vi "VIH HelpGen - HTML - Build A HREF Tag to File.vi"(7 "HTML Folder":path, 8 "file status":enum16{"unknown", "good", "bad"}(ring), 10 "Referenced HTML File":path, 11 "Name":string) -> (0 "file status out":enum16{"unknown", "good", "bad"}(ring), 2 "dup Referenced HTML File":path, 3 "HTML out":string)   [LabVIEW 2014]
doc: "::: VI Helpeks :::\nCopyright (c) 2000-2026 Konstantin Shifershteyn. All rights reserved."
panel:
  # "VI Helpeks\nCopyright (c) 2012-2026 Konstantin Shifershteyn"
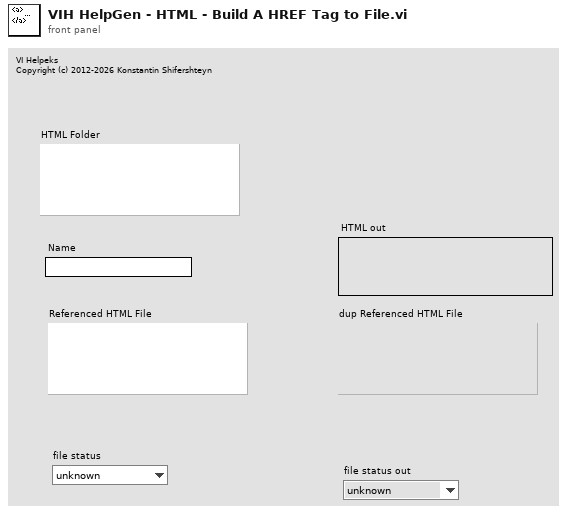
[diagram p1: front panel]
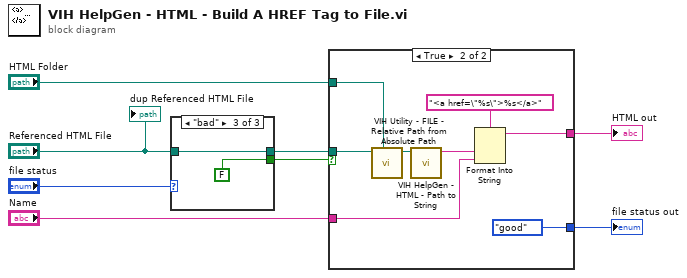
[diagram p0: block diagram]
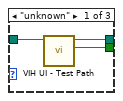
[diagram p2: hidden frame]
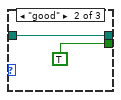
[diagram p3: hidden frame]
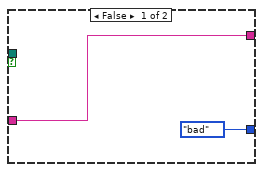
[diagram p4: hidden frame]
diagram:
  n1 = case shown="\"bad\"" "file status" {
    tunnel: "Referenced HTML File" -> [w11 w13 w15]
    tunnel: [w10 w13 w15] -> w6
    tunnel: [w9 TRUE FALSE] -> w4
    frame "unknown" {
      n2 = call "VIH UI - Test Path.vi"("Path"=w11) -> ("Good Path"=w9:bool, "dup Path"=w10:path)  [unwired: 7 in, 2 out]
    }
    frame "good" {
    }
    frame "bad" {
    }
  }
  n3 = case shown="True" w4 {
    tunnel: "HTML Folder" -> [_ w22]
    tunnel: "Name" -> [w17 w21]
    tunnel: w6 -> [_ w20]
    tunnel: [w17 w19] -> w5
    tunnel: [enum16{"unknown", "good", "bad"}."bad" ("file status out") enum16{"unknown", "good", "bad"}."good" ("file status out")] -> w2
    frame False {
    }
    frame True {
      n4 = call "VIH Utility - FILE - Relative Path from Absolute Path.vi"("base path (empty: dir of Top VI)"=w22, "Path"=w20) -> ("Rel Path out"=w24:path)  [unwired: 7 in, 2 out]
      n5 = call "VIH HelpGen - HTML - Path to String.vi"("Path"=w24) -> ("String"=w25:string)  [unwired: 10 in]
      n6 = Format Into String(format string="<a href=\"%s\">%s</a>", w25, w21) -> (resulting string=w19:string)  [unwired: 2 in, 1 out]
    }
  }
  "HTML out" <- w5
  "file status out" <- w2
  "dup Referenced HTML File" <- "Referenced HTML File"
